vi "onComputeIntervals.vi"(8 "error in (no error)":errorcluster, 9 "Cron Interval":T1, 10 "Expression":string, 11 "Cron.Jenkins in":refnum<class "Cron.Jenkins.lvclass">) -> (0 "error out":errorcluster, 2 "Interval Parameters":T2, 3 "Cron.Jenkins out":refnum<class "Cron.Jenkins.lvclass">)   [LabVIEW 2013, in "openCron.lvlib" / "Cron.Jenkins.lvclass"]
uses:
  Cron.Jenkins.lvclass
  Cron/Cron Interval -- cluster.ctl
  Cron/Cron Interval -- enum.ctl
  Cron.Jenkins.lvclass/Cron.Jenkins.ctl
  <vilib>/Utility/MD5Checksum.llb/MD5Checksum string.vi
  Cron/Cron.lvclass
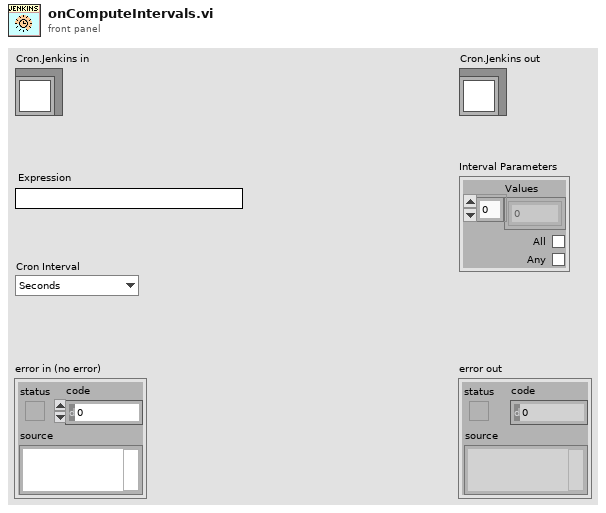
[diagram p1: front panel]
types:
  T1 = typedef "openCron.lvlib/Cron.lvclass/Cron Interval -- enum.ctl" = enum16{"Seconds", "Minutes", "Hours", "Day of Month", "Month", "Day of Week", "Year"}
  T2 = typedef "openCron.lvlib/Cron.lvclass/Cron Interval -- cluster.ctl" = cluster{"Values":i32[], "All":bool, "Any":bool}
  T3 = enum16{"SUN", "MON", "TUE", "WED", "THU", "FRI", "SAT"}
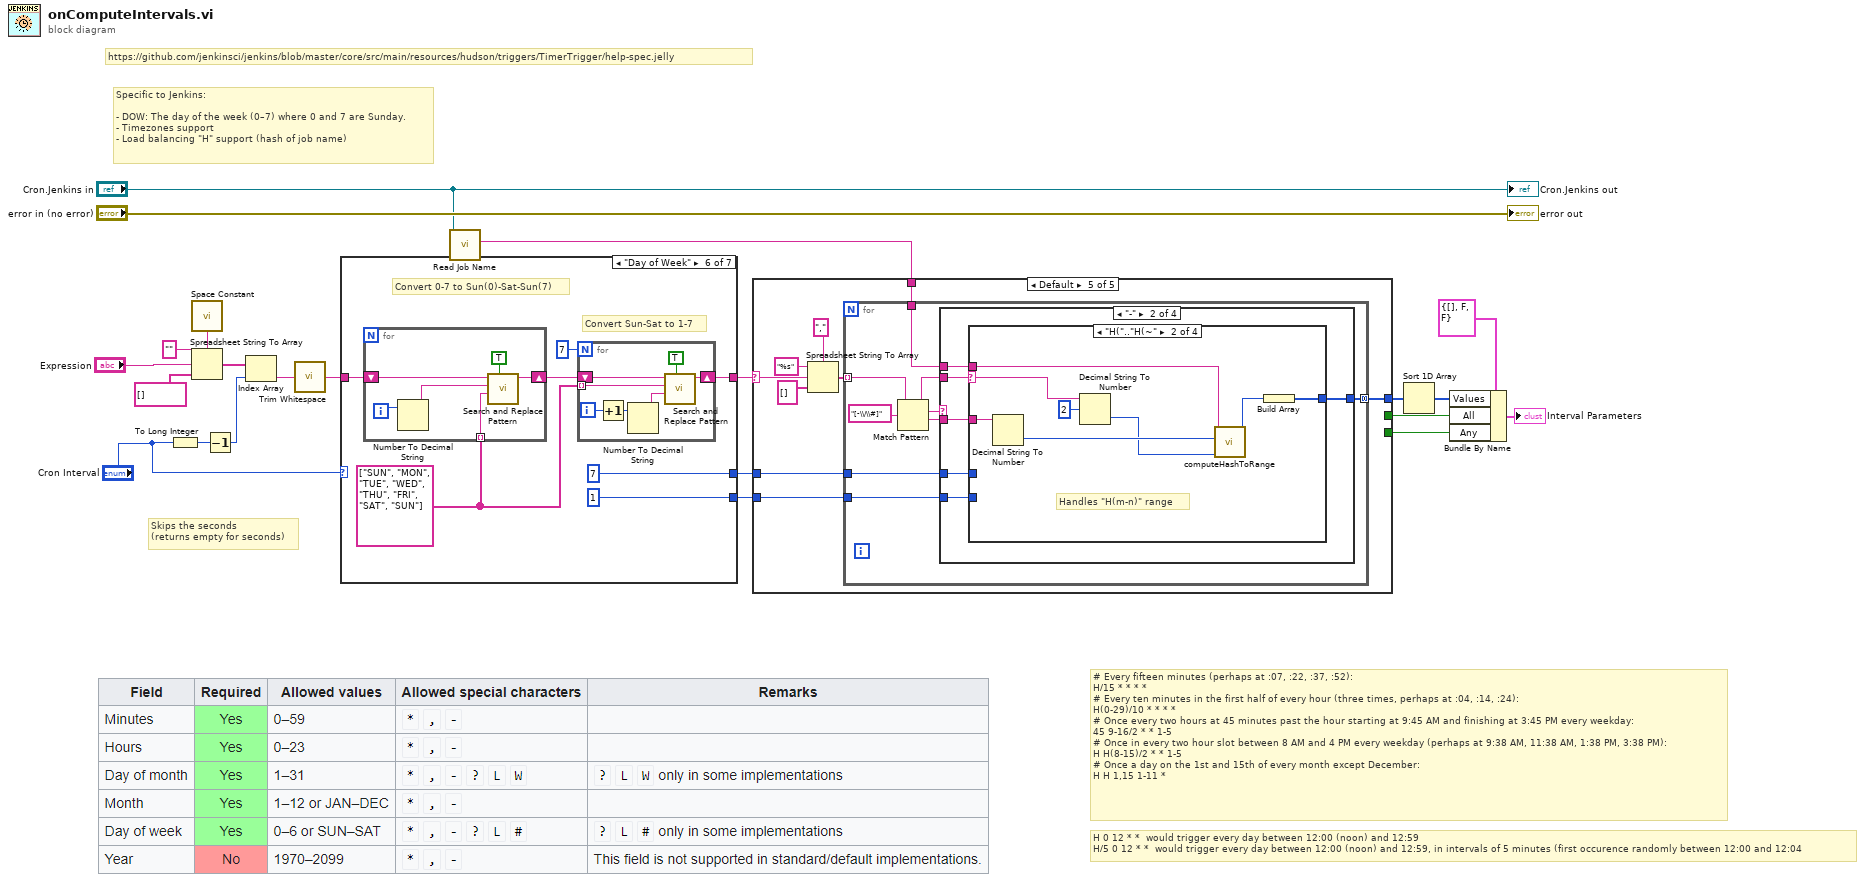
[diagram p0: block diagram]
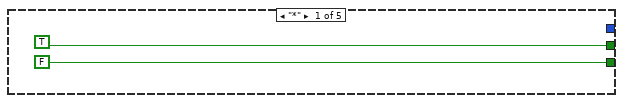
[diagram p2: hidden frame]
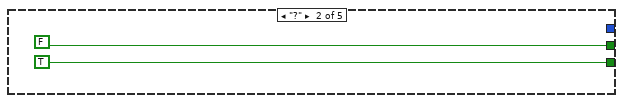
[diagram p3: hidden frame]
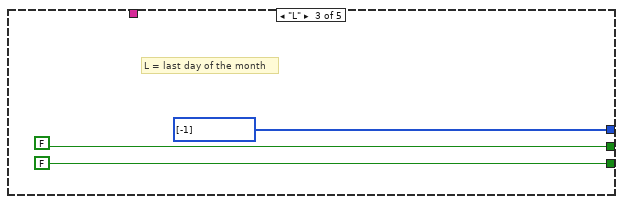
[diagram p4: hidden frame]
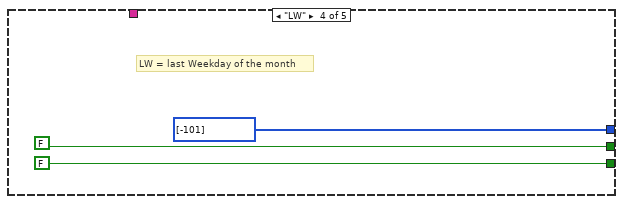
[diagram p5: hidden frame]
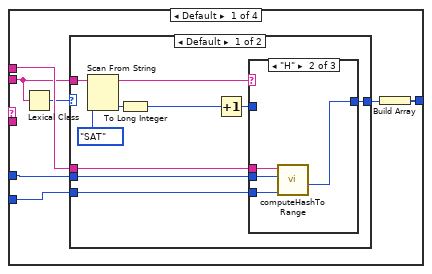
[diagram p6: hidden frame]
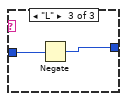
[diagram p8: hidden frame]
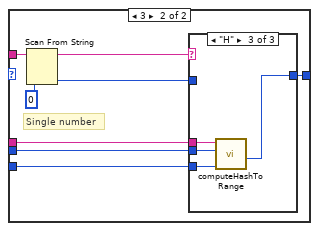
[diagram p9: hidden frame]
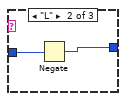
[diagram p11: hidden frame]
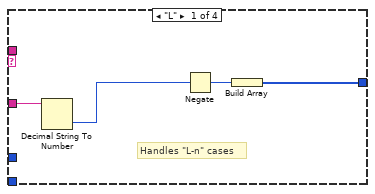
[diagram p12: hidden frame]
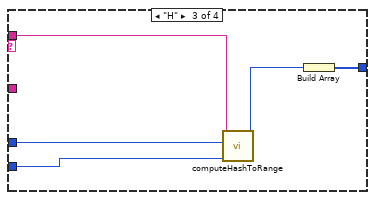
[diagram p13: hidden frame]
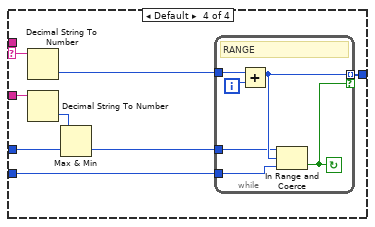
[diagram p14: hidden frame]
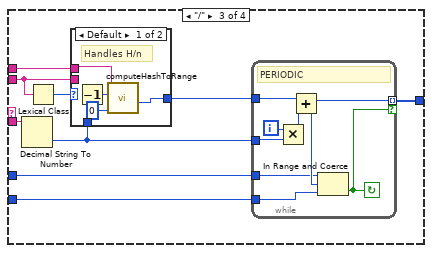
[diagram p15: hidden frame]
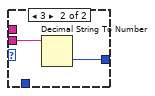
[diagram p16: hidden frame]
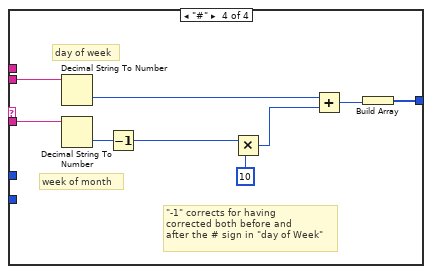
[diagram p17: hidden frame]
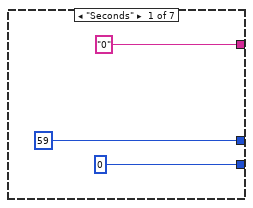
[diagram p18: hidden frame]
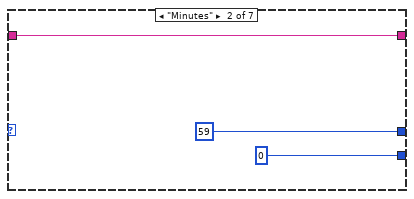
[diagram p19: hidden frame]
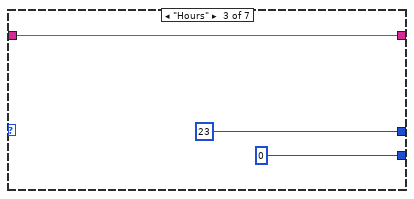
[diagram p20: hidden frame]
diagram:
  # "Skips the seconds\n(returns empty for seconds)"
  # "# Every fifteen minutes (perhaps at :07, :22, :37, :52):\nH/15 * * * *\n# Every ten minutes in the first half of every hour (three times, perhaps at :04, :14, :24):\nH(0-29)/10 * * * *\n# Once every two hours at 45 minutes past the hour starting at 9:45 AM and finishing at 3:45 PM every weekday:\n45 9-16/2 * * 1-5\n# Once in every two hour slot between 8 AM and 4 PM every weekday (perhaps at 9:38 AM, 11:38 AM, 1:38 PM, 3:38 PM):\nH H(8-15)/2 * * 1-5\n# Once a day on the 1st and 15th of every month except December:\nH H 1,15 1-11 *"
  # "Specific to Jenkins: \n\n- DOW: The day of the week (0–7) where 0 and 7 are Sunday.\n- Timezones support\n- Load balancing \"H\" support (hash of job name)"
  # "https://github.com/jenkinsci/jenkins/blob/master/core/src/main/resources/hudson/triggers/TimerTrigger/help-spec.jelly"
  # "H 0 12 * *  would trigger every day between 12:00 (noon) and 12:59\nH/5 0 12 * *  would trigger every day between 12:00 (noon) and 12:59, in intervals of 5 minutes (first occurence randomly between 12:00 and 12:04"
  n1 = To Long Integer(number="Cron Interval") -> (32bit integer=w4:i32)
  n2 = call <vilib>:"Space Constant.vi"() -> ("String"=w16:string)
  n3 = Spreadsheet String To Array(delimiter (Tab)=w16, format string="", spreadsheet string="Expression", array type (2D Dbl)=string[] []) -> (array=w15:string[])
  n4 = Decrement(x=w4) -> (x-1=w3:i32)
  n5 = Index Array(array=w15, index=w3) -> (element=w14:string)
  n6 = call <vilib>:"Trim Whitespace.vi"("string"=w14) -> ("trimmed string"=w6:string)  [unwired: 1 in]
  n7 = case shown="\"Day of Week\"" "Cron Interval" {
    tunnel: [59 ("y") 59 ("y") 23 ("y") 31 ("y") 12 ("y") 7 ("y") 2099 ("y")] -> w13
    tunnel: [0 ("y") 0 ("y") 0 ("y") 1 ("y") 1 ("y") 1 ("y") 1970 ("y")] -> w12
    tunnel: w6 -> [_ w26 w29 w32 w36 w50 w67]
    tunnel: ["0" ("trimmed string") w26 w29 w32 w37 w51 w67] -> w5
    frame "Seconds" {
    }
    frame "Minutes" {
    }
    frame "Hours" {
    }
    frame "Day of Month" {
    }
    frame "Month" {
      n8 = for {
        shift-right: [w46] -> w37
        shift-left: w36 -> [w45]
        tunnel: string[] ["JAN", "FEB", "MAR", "APR", "MAY", "JUN", "JUL", "AUG", "SEP", "OCT", "NOV", "DEC"] -> [w43] mode=indexing
        i -> [w42]
        n9 = Increment(x=w42) -> (x+1=w41:i32)
        n10 = Number To Decimal String(number=w41) -> (decimal integer string=w40:string)  [unwired: 1 in]
        n11 = call <vilib>:"Search and Replace Pattern.vi"("string"=w45, "regular expression (\"\")"=w43, "replace string (\"\")"=w40, "replace all? (F)"=TRUE) -> ("result string"=w46:string)  [unwired: 1 in, 1 out]
      }
    }
    frame "Day of Week" {
      w48 = string[] ["SUN", "MON", "TUE", "WED", "THU", "FRI", "SAT", "SUN"]
      # "Convert Sun-Sat to 1-7"
      # "Convert 0-7 to Sun(0)-Sat-Sun(7)"
      n12 = for {
        shift-right: [w59] -> w49
        shift-left: w50 -> [w58]
        tunnel: w48 -> [w56] mode=indexing
        i -> [w55]
        n13 = Number To Decimal String(number=w55) -> (decimal integer string=w54:string)  [unwired: 1 in]
        n14 = call <vilib>:"Search and Replace Pattern.vi"("string"=w58, "regular expression (\"\")"=w54, "replace string (\"\")"=w56, "replace all? (F)"=TRUE) -> ("result string"=w59:string)  [unwired: 1 in, 1 out]
      }
      n15 = for {
        N: 7 -> [_]
        shift-right: [w66] -> w51
        shift-left: w49 -> [w65]
        tunnel: w48 -> [w63] mode=indexing
        i -> [w61]
        n16 = Increment(x=w61) -> (x+1=w60:i32)
        n17 = Number To Decimal String(number=w60) -> (decimal integer string=w62:string)  [unwired: 1 in]
        n18 = call <vilib>:"Search and Replace Pattern.vi"("string"=w65, "regular expression (\"\")"=w63, "replace string (\"\")"=w62, "replace all? (F)"=TRUE) -> ("result string"=w66:string)  [unwired: 1 in, 1 out]
      }
    }
    frame "Year" {
    }
  }
  n19 = call "Read Job Name.vi"("Cron.Jenkins in"="Cron.Jenkins in") -> ("Job Name"=w1:string)  [unwired: 8 in, 2 out]
  n20 = case shown="Default" w5 {
    selector: w5 -> [_ _ _ _ w84]
    tunnel: [_ _ i32[] [-1] i32[] [-101] w83] -> w10
    tunnel: [TRUE FALSE FALSE FALSE _] -> w9
    tunnel: [FALSE TRUE FALSE FALSE _] -> w8
    tunnel: w13 -> [_ _ _ _ w82]
    tunnel: w12 -> [_ _ _ _ w81]
    tunnel: w1 -> [_ _ _ _ w80]
    frame "*" {
    }
    frame "?" {
    }
    frame "L" {
      # "L = last day of the month"
    }
    frame "LW" {
      # "LW = last Weekday of the month"
    }
    frame Default {
      n21 = Spreadsheet String To Array(delimiter (Tab)=",", format string="%s", spreadsheet string=w84, array type (2D Dbl)=string[] []) -> (array=w85:string[])
      n22 = for {
        tunnel: w85 -> [w97] mode=indexing
        tunnel: [w93] -> w83 mode=concatenating
        tunnel: w82 -> [w91]
        tunnel: w81 -> [w90]
        tunnel: w80 -> [w89]
        n23 = Match Pattern(string=w97, regular expression="[-\\/\\#]") -> (before substring=w94:string, match substring=w95:string, after substring=w92:string)  [unwired: 1 in, 1 out]
        n24 = case shown="\"-\"" w95 {
          tunnel: w94 -> [w99 w138 w176 w206]
          tunnel: [w104 w141 w182 w204] -> w93
          tunnel: w92 -> [_ w142 w181 w205]
          tunnel: w91 -> [w102 w140 w180 _]
          tunnel: w90 -> [w101 w139 w179 _]
          tunnel: w89 -> [w100 w137 w174 _]
          frame Default {
            n25 = Lexical Class(1:w99) -> (0:w98:i16)
            n26 = case shown="Default" w98 {
              tunnel: [w108 w127] -> w103
              tunnel: w99 -> [w114 w129]
              tunnel: w100 -> [w107 w124]
              tunnel: w102 -> [w106 w123]
              tunnel: w101 -> [w105 w122]
              frame Default {
                n27 = Scan From String(input string=w114, default 1=T3."SAT" ("y")) -> (remaining string=w110:string, output 1=w111:T3)  [unwired: 3 in, 2 out]
                n28 = To Long Integer(number=w111) -> (32bit integer=w112:i32)
                n29 = Increment(x=w112) -> (x+1=w109:i32)
                n30 = case shown="\"H\"" w110 {
                  tunnel: w109 -> [w115 _ w121]
                  tunnel: [w115 w116 w120] -> w108
                  tunnel: w107 -> [_ w119 _]
                  tunnel: w106 -> [_ w118 _]
                  tunnel: w105 -> [_ w117 _]
                  frame Default {
                  }
                  frame "H" {
                    n31 = call "computeHashToRange.vi"("min Value"=w117, "maxValue"=w118, "seed"=w119) -> ("H"=w116:i32)  [unwired: 8 in]
                  }
                  frame "L" {
                    n32 = Negate(x=w121) -> (-x=w120:i32)
                  }
                }
              }
              frame 3 {
                # "Single number"
                n33 = Scan From String(input string=w129, default 1=0 ("32bit integer")) -> (remaining string=w128:string, output 1=w125:i32)  [unwired: 3 in, 2 out]
                n34 = case shown="\"H\"" w128 {
                  tunnel: w125 -> [w130 w132 _]
                  tunnel: [w130 w131 w133] -> w127
                  tunnel: w124 -> [_ _ w136]
                  tunnel: w123 -> [_ _ w135]
                  tunnel: w122 -> [_ _ w134]
                  frame Default {
                  }
                  frame "L" {
                    n35 = Negate(x=w132) -> (-x=w131:i32)
                  }
                  frame "H" {
                    n36 = call "computeHashToRange.vi"("min Value"=w134, "maxValue"=w135, "seed"=w136) -> ("H"=w133:i32)  [unwired: 8 in]
                  }
                }
              }
            }
            n37 = Build Array(w103) -> (w104:i32[])
          }
          frame "-" {
            n38 = case shown="\"H(\"..\"H(~\"" w138 {
              selector: w138 -> [_ w149 _ w160]
              tunnel: w142 -> [w146 w151 _ w166]
              tunnel: [w144 w154 w159 w165] -> w141
              tunnel: w140 -> [_ _ w158 w163]
              tunnel: w139 -> [_ _ w157 w162]
              tunnel: w137 -> [_ w153 w156 _]
              frame "L" {
                # "Handles \"L-n\" cases"
                n39 = Decimal String To Number(string=w146) -> (number=w145:i32)  [unwired: 2 in, 1 out]
                n40 = Negate(x=w145) -> (-x=w143:i32)
                n41 = Build Array(w143) -> (w144:i32[])
              }
              frame "H(".."H(~" {
                # "Handles \"H(m-n)\" range"
                n42 = Decimal String To Number(string=w151) -> (number=w150:i32)  [unwired: 2 in, 1 out]
                n43 = Decimal String To Number(string=w149, offset=2) -> (number=w147:i32)  [unwired: 1 in, 1 out]
                n44 = call "computeHashToRange.vi"("min Value"=w147, "maxValue"=w150, "seed"=w153) -> ("H"=w152:i32)  [unwired: 8 in]
                n45 = Build Array(w152) -> (w154:i32[])
              }
              frame "H" {
                n46 = call "computeHashToRange.vi"("min Value"=w157, "maxValue"=w158, "seed"=w156) -> ("H"=w155:i32)  [unwired: 8 in]
                n47 = Build Array(w155) -> (w159:i32[])
              }
              frame Default {
                n48 = Decimal String To Number(string=w160) -> (number=w167:i32)  [unwired: 2 in, 1 out]
                n49 = Decimal String To Number(string=w166) -> (number=w164:i32)  [unwired: 2 in, 1 out]
                n50 = Max & Min(x=w164, y=w163) -> (min(x,y)=w161:i32)  [unwired: 1 out]
                n51 = while {
                  tunnel: w167 -> [w173]
                  tunnel: [w170] -> w165 mode=indexing if=w171
                  tunnel: w162 -> [w169]
                  tunnel: w161 -> [w168]
                  i -> [w172]
                  stop <- w171 continue-if-true
                  # "RANGE"
                  n52 = Add(x=w173, y=w172) -> (x+y=w170:i32)
                  n53 = In Range and Coerce(upper limit=w168, x=w170, lower limit=w169) -> (In Range?=w171:bool)  [unwired: 1 out]
                }
              }
            }
          }
          frame "/" {
            n54 = Decimal String To Number(string=w181) -> (number=w177:i32)  [unwired: 2 in, 1 out]
            n55 = Lexical Class(1:w176) -> (0:w178:i16)
            n56 = case shown="Default" w178 {
              tunnel: [w185 w189] -> w175
              tunnel: w176 -> [_ w188]
              tunnel: w174 -> [w183 _]
              tunnel: w177 -> [w187 _]
              frame Default {
                # "Handles H/n"
                n57 = Decrement(x=w187) -> (x-1=w184:i32)
                n58 = call "computeHashToRange.vi"("min Value"=0, "maxValue"=w184, "seed"=w183) -> ("H"=w185:i32)  [unwired: 8 in]
              }
              frame 3 {
                n59 = Decimal String To Number(string=w188) -> (number=w189:i32)  [unwired: 2 in, 1 out]
              }
            }
            n60 = while {
              tunnel: w175 -> [w197]
              tunnel: [w193] -> w182 mode=indexing if=w190
              tunnel: w177 -> [w196]
              tunnel: w180 -> [w192]
              tunnel: w179 -> [w191]
              i -> [w195]
              stop <- w190 continue-if-true
              # "PERIODIC"
              n61 = Multiply(x=w195, y=w196) -> (x*y=w194:i32)
              n62 = Add(x=w197, y=w194) -> (x+y=w193:i32)
              n63 = In Range and Coerce(upper limit=w192, x=w193, lower limit=w191) -> (In Range?=w190:bool)  [unwired: 1 out]
            }
          }
          frame "#" {
            # "\"-1\" corrects for having\ncorrected both before and\nafter the # sign in \"day of Week\""
            # "week of month"
            # "day of week"
            n64 = Decimal String To Number(string=w206) -> (number=w200:i32)  [unwired: 2 in, 1 out]
            n65 = Decimal String To Number(string=w205) -> (number=w203:i32)  [unwired: 2 in, 1 out]
            n66 = Decrement(x=w203) -> (x-1=w198:i32)
            n67 = Multiply(x=w198, y=10) -> (x*y=w199:i32)
            n68 = Add(x=w200, y=w199) -> (x+y=w201:i32)
            n69 = Build Array(w201) -> (w204:i32[])
          }
        }
      }
    }
  }
  n70 = Sort 1D Array(array=w10) -> (sorted array=w11:i32[])
  n71 = Bundle By Name(cluster=T2 {"Values"=[], "All"=FALSE, "Any"=FALSE} ("Interval"), "Values"=w11, "All"=w9, "Any"=w8) -> (→"Interval Parameters":T2)
  "error out" <- "error in (no error)"
  "Cron.Jenkins out" <- "Cron.Jenkins in"
